vi "SC Ask Robot.vi"() -> (1 "address":string, 2 "ok?":bool)   [LabVIEW 2023]
doc: "Asks for a robot's address (name or IP). Returns it, or ok? = false when the user cancels or closes the window."
uses:
  <vilib>/Utility/error.llb/Trim Whitespace One-Sided.vi
panel:
  in  "Cancel":bool
  in  "OK":bool
  in  "Robot address (name or IP)":string="robot.local"
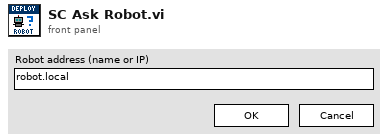
[diagram p1: front panel]
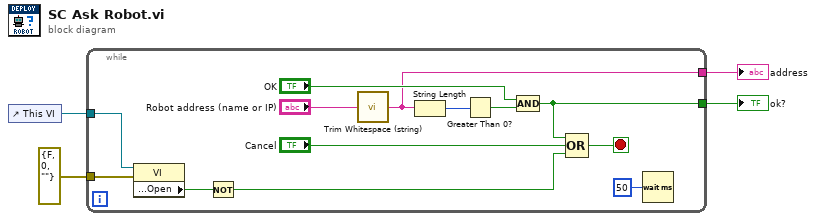
[diagram p0: block diagram]
diagram:
  n1 = control-ref of="This VI"() -> (w4:refnum<vi>)
  n2 = while {
    tunnel: w4 -> [w17]
    tunnel: errorcluster {"status"=FALSE, "code"=0, "source"=""} -> [w16]
    tunnel: [w6] -> w2
    tunnel: [w5] -> w1
    stop <- w7 stop-if-true
    n3 = property class="VI"(reference=w17, error in=w16) -> ("Front Panel Window:Open"=w15:bool)  [unwired: 2 out]
    n4 = Not(x=w15) -> (.not. x?=w9:bool)
    n5 = call <vilib>:"Trim Whitespace (string).vi"("string"="Robot address (name or IP)") -> ("trimmed string"=w6:string)  [unwired: 1 in]
    n6 = String Length(string=w6) -> (length=w13:i32)
    n7 = Greater Than 0?(x=w13) -> (x > 0?=w11:bool)
    n8 = Compound Arithmetic op=AND("OK", w11) -> (w5:bool)
    n9 = Compound Arithmetic op=OR(w5, "Cancel", w9) -> (w7:bool)
    n10 = Wait (ms)(milliseconds to wait=50) -> ()  [unwired: 1 out]
  }
  "address" <- w2
  "ok?" <- w1
